vi "lvmcp_gen_script.vi"() -> ()   [LabVIEW 2015]
panel:
  in  "Data Strings":string[](array[string])
  in  "Type Strings":string[](array[string])
  in  "Obj Refs In[]":refnum<vi>[](array[refnum])
  out "error out":errorcluster
  out "Obj Refs Out[]":refnum<vi>[](array[refnum])
  in  "XML Script Commands":string
  in  "reference":refnum<vi>
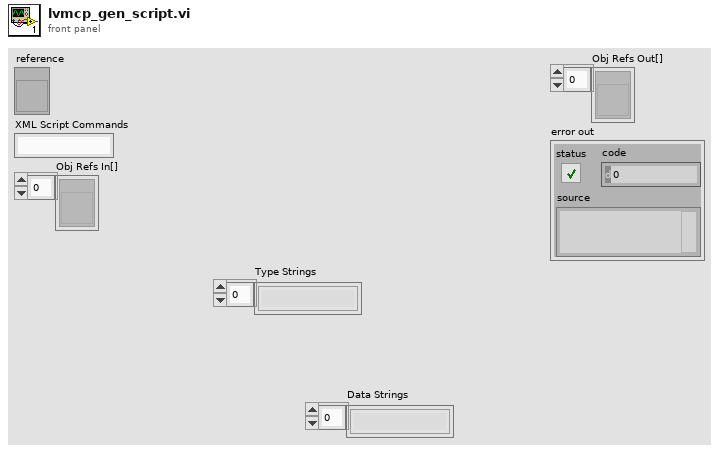
[diagram p1: front panel]
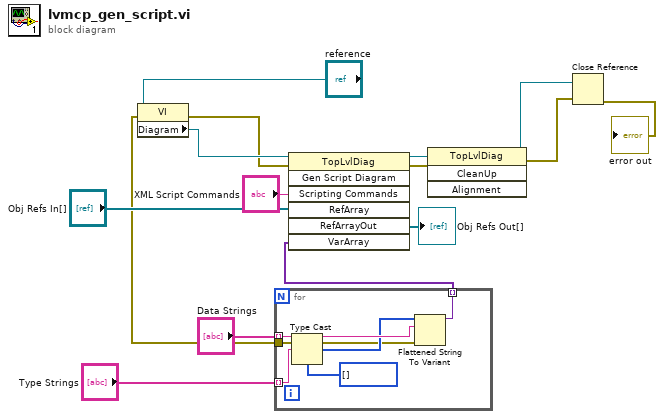
[diagram p0: block diagram]
diagram:
  n1 = for {
    tunnel: "Type Strings" -> [w20] mode=indexing
    tunnel: "Data Strings" -> [w19] mode=indexing
    tunnel: [w17] -> w6 mode=indexing
    tunnel: [w16] -> w5
    n2 = Type Cast(type=i16[] [] ("type string"), x=w20) -> (*(type *) &x=w18:i16[])
    n3 = Flattened String To Variant(6:w19, 7:w18) -> (0:w16:errorcluster, 3:w17:variant)  [unwired: 1 in]
  }
  n4 = property class="VI"(reference="reference", error in=w5) -> (error out=w13:errorcluster, "Diagram"=w14:refnum<vi>)  [unwired: 1 out]
  n5 = invoke class="TopLvlDiag" method="Gen Script Diagram"(reference=w14, error in=w13, "Scripting Commands"="XML Script Commands", "RefArray"="Obj Refs In[]", "VarArray"=w6) -> (reference out=w4:refnum<vi>, error out=w3:errorcluster, "RefArrayOut"=→"Obj Refs Out[]":refnum<vi>[])  [unwired: 2 in, 4 out]
  n6 = invoke class="TopLvlDiag" method="CleanUp"(reference=w4, error in=w3) -> (reference out=w2:refnum<vi>, error out=w1:errorcluster)  [unwired: 2 in, 2 out]
  n7 = Close Reference(reference=w2, error in (no error)=w1) -> (error out=→"error out":errorcluster)
